vi "Read Graph Axis Labels (UTF-8 String).vi"(8 "error in":errorcluster, 11 "Control Ref":refnum<vi>) -> (0 "error out":errorcluster, 1 "Y Axis":refnum<class "UTF-8 String.lvclass">, 2 "X Axis":refnum<class "UTF-8 String.lvclass">)   [LabVIEW 2020, in "G-Unicode.lvlib"]
doc: "Read unicode text from a control or text element of a control. If the control text is not unicode, it will be converted to unicode."
uses:
  G-Unicode.lvlib
  Types/UTF-8 String/UTF-8 String.lvclass
  Types/UTF-8 String/UTF-8 String.lvclass/UTF-8 String.ctl
  f6f7f231-7ddf-476b-a943-0386d848a5c9.vi
  3fa1dd17-8c9f-4d8d-ac67-ec21dd2df23f.vi
  Types/UTF-8 String/New UTF-8 String.vi
  Unicode/Encode String.vi
  Private/Conversion/Text to UTF-8.vi
  Private/Conversion/Polymorphic VIs/Text to UTF-8 (LabVIEW String).vi
  Private/Conversion/Encoded UTF-8 String to Encoded UTF-16LE String.vi
  Unicode/SubVIs/UTF-16 Byte Swap.vi
  Private/Conversion/UTF-8 to Text.vi
  Private/Conversion/Polymorphic VIs/UTF-8 to Text (LabVIEW String).vi
  Private/Conversion/Encoded UTF-16LE String to Encoded UTF-8 String.vi
  Unicode/Prepend BOM.vi
  Unicode/SubVIs/Byte Order Marks.vi
  Unicode/Detect BOM.vi
  Unicode/Detect String Encoding.vi
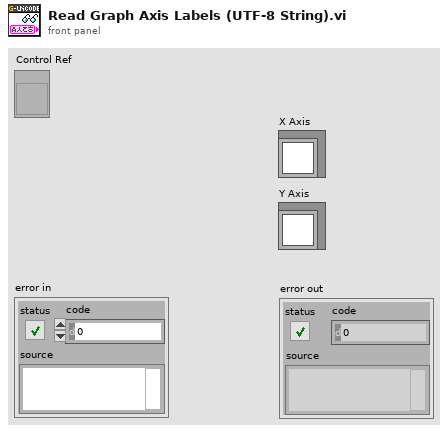
[diagram p1: front panel]
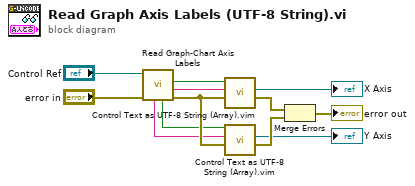
[diagram p0: block diagram]
diagram:
  n1 = call "Read Graph-Chart Axis Labels.vi"("error in"="error in", "Graph / Chart Reference in"="Control Ref") -> ("error out"=w7:errorcluster, "X Axis"=w9:string, "Interpret As Unicode (X)"=w10:bool, "Interpret As Unicode (Y)"=w5:bool, "Y Axis"=w6:string)  [unwired: 4 in, 1 out]
  n2 = call "Control Text as UTF-8 String (Array).vim"("Interpret As Unicode"=w10, "error in"=w7, "Control Text"=w9) -> ("error out"=w3:errorcluster, "UTF-8 String"=→"X Axis":refnum<class "UTF-8 String.lvclass">)  [unwired: 7 in]
  n3 = call "Control Text as UTF-8 String (Array).vim"("Interpret As Unicode"=w5, "error in"=w7, "Control Text"=w6) -> ("error out"=w4:errorcluster, "UTF-8 String"=→"Y Axis":refnum<class "UTF-8 String.lvclass">)  [unwired: 7 in]
  n4 = Merge Errors(w3, w4) -> (→"error out":errorcluster)
